vi "Search Fundamental Frequency.vi"(8 "error in (no error)":errorcluster caption="에러 입력(에러 없음)", 10 "Center Frequency (Hz)":dbl, 11 "Instrument Manager 입력":refnum<class "Instrument Manager.lvclass">) -> (0 "error out":errorcluster caption="에러 출력", 2 "Marker Value":T1 {"X-axis" format="%#_6p"}, 3 "Instrument Manager 출력":refnum<class "Instrument Manager.lvclass">)   [LabVIEW 2023, in "Instrument Manager.lvclass"]
uses:
  Instrument Manager.lvclass
  Module/Spectrum Analyzer/TYPE DEFINITION/TYPE Marker Value.ctl
  Module/Spectrum Analyzer/TYPE DEFINITION/TYPE Detect Mode Select.ctl
  Module/Spectrum Analyzer/TYPE DEFINITION/TYPE Display Trace Mode Select.ctl
  8293ca82-960d-42ec-acc2-4c2ddc49d3c3.vi
  ae7db660-397e-4acb-8eee-160e082d7eae.vi
  d05fff4c-afac-49ab-a027-b280e4e3bd07.vi
  Instrument Manager.lvclass/Instrument Manager.ctl
  Module/Spectrum Analyzer/Spectrum Analyzer.lvlib
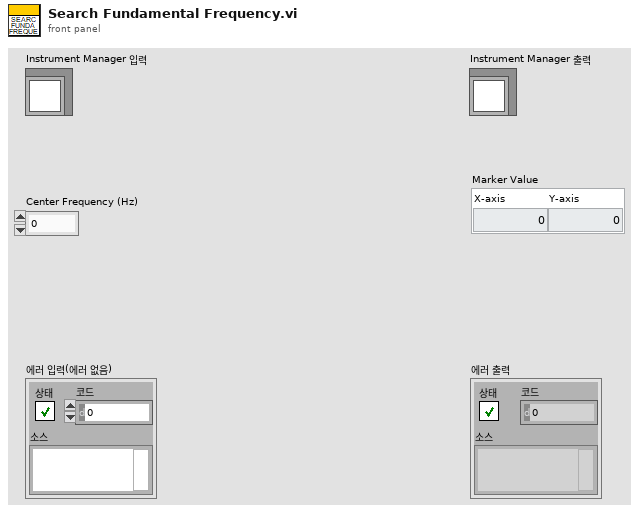
[diagram p1: front panel]
types:
  T1 = typedef "Spectrum Analyzer.lvlib/TYPE Marker Value.ctl" = cluster{"X-axis":dbl, "Y-axis":dbl}
  T2 = typedef "Spectrum Analyzer.lvlib/TYPE Display Trace Mode Select.ctl" = enum16{"Clear Write", "Max Hold", "Min Hold", "Average", "View"}
  T3 = typedef "Spectrum Analyzer.lvlib/TYPE Detect Mode Select.ctl" = enum16{"Det Auto (Normal)", "Auto Peak", "Positive Peak", "Negative Peak", "Sample", "RMS", "Average", "Quasipeak", "CISPR Average", "RMS Average"}
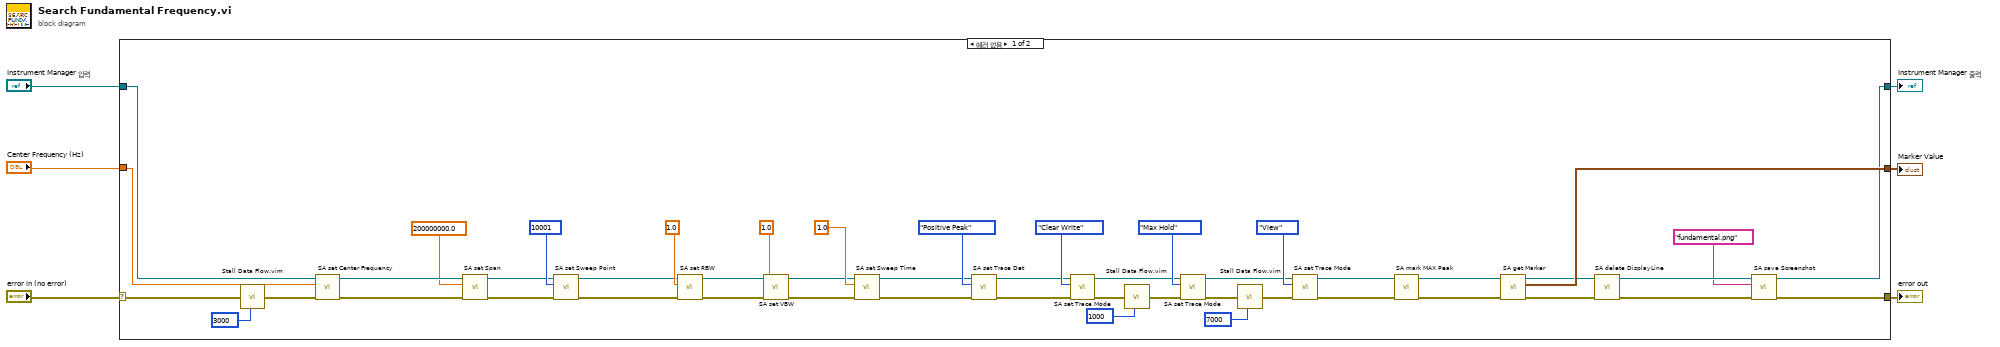
[diagram p0: block diagram]
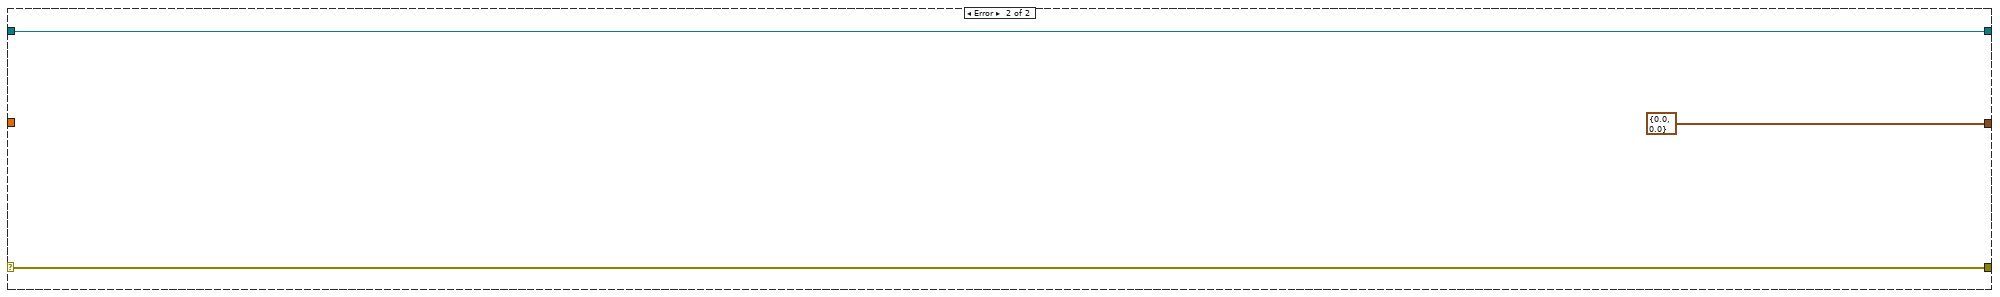
[diagram p2: hidden frame]
diagram:
  n1 = case shown="에러 없음" "error in (no error)" {
    selector: "error in (no error)" -> [w13 w57]
    tunnel: [w9 w57] -> w5
    tunnel: [w8 w56] -> w3
    tunnel: "Instrument Manager 입력" -> [w35 w56]
    tunnel: "Center Frequency (Hz)" -> [w48 _]
    tunnel: [w24 T1 {"X-axis"=0.0, "Y-axis"=0.0} ("Marker Value")] -> w1
    frame No Error {
      n2 = call "Stall Data Flow.vim"("value in"=w13, "milliseconds to wait"=u32 3000) -> ("value out"=w12:errorcluster)  [unwired: 1 out]
      n3 = call "SA set Center Frequency.vi"("error in (no error)"=w12, "Center Frequency (Hz)"=w48, "Instrument Manager 입력"=w35) -> ("error out"=w21:errorcluster, "Instrument Manager 출력"=w19:refnum<class "Instrument Manager.lvclass">)  [unwired: 7 in]
      n4 = call "SA set Span.vi"("error in (no error)"=w21, "Span (Hz)"=200000000.0, "Instrument Manager 입력"=w19) -> ("error out"=w20:errorcluster, "Instrument Manager 출력"=w18:refnum<class "Instrument Manager.lvclass">)  [unwired: 7 in]
      n5 = call "SA set Sweep Point.vi"("error in (no error)"=w20, "Sweep Point"=u32 10001, "Instrument Manager 입력"=w18) -> ("error out"=w54:errorcluster, "Instrument Manager 출력"=w34:refnum<class "Instrument Manager.lvclass">)  [unwired: 7 in]
      n6 = call "SA set RBW.vi"("error in (no error)"=w54, "BW Value (Hz)"=1.0, "Instrument Manager 입력"=w34) -> ("error out"=w53:errorcluster, "Instrument Manager 출력"=w33:refnum<class "Instrument Manager.lvclass">)  [unwired: 7 in]
      n7 = call "SA set VBW.vi"("error in (no error)"=w53, "BW Value (Hz)"=1.0, "Instrument Manager 입력"=w33) -> ("error out"=w52:errorcluster, "Instrument Manager 출력"=w32:refnum<class "Instrument Manager.lvclass">)  [unwired: 7 in]
      n8 = call "SA set Sweep Time.vi"("error in (no error)"=w52, "Sweep Time(sec)"=1.0, "Instrument Manager 입력"=w32) -> ("error out"=w51:errorcluster, "Instrument Manager 출력"=w31:refnum<class "Instrument Manager.lvclass">)  [unwired: 7 in]
      n9 = call "SA set Trace Det.vi"("error in (no error)"=w51, "Detector Type"=TYPE_Detect_Mode_Select."Positive Peak", "Instrument Manager 입력"=w31) -> ("error out"=w50:errorcluster, "Instrument Manager 출력"=w30:refnum<class "Instrument Manager.lvclass">)  [unwired: 7 in]
      n10 = call "SA set Trace Mode.vi"("error in (no error)"=w50, "Trace Mode"=TYPE_Display_Trace_Mode_Select."Clear Write", "Instrument Manager 입력"=w30) -> ("error out"=w39:errorcluster, "Instrument Manager 출력"=w29:refnum<class "Instrument Manager.lvclass">)  [unwired: 7 in]
      n11 = call "Stall Data Flow.vim"("value in"=w39, "milliseconds to wait"=u32 1000) -> ("value out"=w38:errorcluster)  [unwired: 1 out]
      n12 = call "SA set Trace Mode.vi"("error in (no error)"=w38, "Trace Mode"=TYPE_Display_Trace_Mode_Select."Max Hold", "Instrument Manager 입력"=w29) -> ("error out"=w37:errorcluster, "Instrument Manager 출력"=w28:refnum<class "Instrument Manager.lvclass">)  [unwired: 7 in]
      n13 = call "Stall Data Flow.vim"("value in"=w37, "milliseconds to wait"=u32 7000) -> ("value out"=w36:errorcluster)  [unwired: 1 out]
      n14 = call "SA set Trace Mode.vi"("error in (no error)"=w36, "Trace Mode"=TYPE_Display_Trace_Mode_Select."View", "Instrument Manager 입력"=w28) -> ("error out"=w26:errorcluster, "Instrument Manager 출력"=w27:refnum<class "Instrument Manager.lvclass">)  [unwired: 7 in]
      n15 = call "SA mark MAX Peak.vi"("error in (no error)"=w26, "Instrument Manager 입력"=w27) -> ("error out"=w49:errorcluster, "Instrument Manager 출력"=w25:refnum<class "Instrument Manager.lvclass">)  [unwired: 8 in]
      n16 = call "SA get Marker.vi"("error in (no error)"=w49, "Instrument Manager 입력"=w25) -> ("error out"=w16:errorcluster, "Marker Value"=w24:T1, "Instrument Manager 출력"=w15:refnum<class "Instrument Manager.lvclass">)  [unwired: 7 in]
      n17 = call "SA delete DisplayLine.vi"("error in (no error)"=w16, "Instrument Manager 입력"=w15) -> ("error out"=w10:errorcluster, "Instrument Manager 출력"=w11:refnum<class "Instrument Manager.lvclass">)  [unwired: 8 in]
      n18 = call "SA save Screenshot.vi"("error in (no error)"=w10, "File Name"="fundamental.png", "Instrument Manager 입력"=w11) -> ("error out"=w9:errorcluster, "Instrument Manager 출력"=w8:refnum<class "Instrument Manager.lvclass">)  [unwired: 7 in]
    }
    frame Error {
    }
  }
  "error out" <- w5
  "Instrument Manager 출력" <- w3
  "Marker Value" <- w1
